vi "libssh2_channel_window_read_ex.vi"(8 "error in (no error)":errorcluster, 11 "channel":T1) -> (0 "error out":errorcluster, 1 "bytes available for read":u32, 2 "initial window size":u32, 3 "remaining read window":u32)   [LabVIEW 2017, in "libssh2.lvlib"]
doc: "Returns the number of bytes which the remote end may send without overflowing the window limit.\n\n<B>bytes available for read</B> returns the number of bytes actually available to be read.\n<B>initial window size</B> returns the initial window size as defined by the channel_open request."
uses:
  libssh2.lvlib
  Channel Refnum.ctl
  Acquire Session.vi
  Release Session.vi
  Not A Channel.vi
  <vilib>/Utility/error.llb/Error Cluster From Error Code.vi
  Global Settings.vi
  Read Channel Refnum.vi
  Read Session Refnum.vi
  <vilib>/Utility/semaphor.llb/Acquire Semaphore.vi
  <vilib>/Utility/semaphor.llb/Release Semaphore.vi
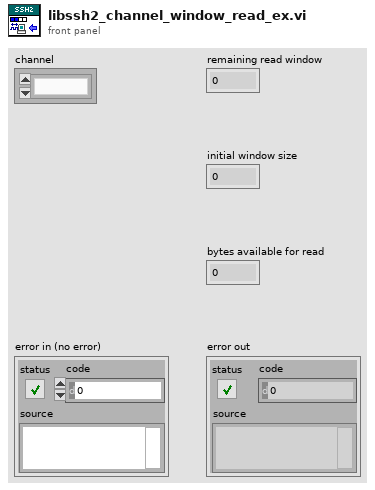
[diagram p1: front panel]
types:
  T1 = typedef "libssh2.lvlib/Channel Refnum.ctl" = refnum<k1>
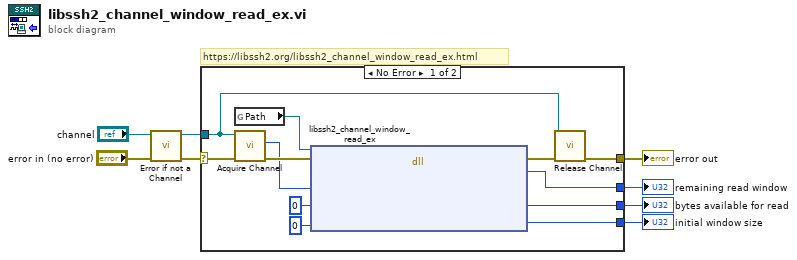
[diagram p0: block diagram]
diagram:
  # "https://libssh2.org/libssh2_channel_window_read_ex.html"
  n1 = call "Error if not a Channel.vi"("error in (no error)"="error in (no error)", "channel"="channel") -> ("error out"=w3:errorcluster, "channel out"=w1:T1)  [unwired: 8 in]
  n2 = case shown="No Error" w3 {
    selector: w3 -> [w20 w21]
    tunnel: [w10 w21] -> w8
    tunnel: w1 -> [w9 _]
    tunnel: [w18 _] -> w6
    tunnel: [w17 _] -> w5
    tunnel: [w16 _] -> w4
    frame No Error {
      n3 = global read "Global Settings.vi" "Path"() -> (w13:path)
      n4 = call "Acquire Channel.vi"("error in (no error)"=w20, "channel"=w9) -> ("error out"=w15:errorcluster, "LIBSSH2_CHANNEL*"=w14:u64)  [unwired: 8 in]
      n5 = dll-call lib="?" fn="libssh2_channel_window_read_ex"(path in=w13, error in=w15, "channel"=w14, "read_avail"=u32 0, "window_size_initial"=u32 0) -> (error out=w19:errorcluster, "return value"=w17:u32, "read_avail"=w16:u32, "window_size_initial"=w18:u32)  [unwired: 2 in, 1 out]
      n6 = call "Release Channel.vi"("error in (no error)"=w19, "channel"=w9) -> ("error out"=w10:errorcluster)  [unwired: 9 in]
    }
    frame Error {
    }
  }
  "error out" <- w8
  "initial window size" <- w6
  "remaining read window" <- w5
  "bytes available for read" <- w4
